vi "Core Read U8 FIFO.vi"(8 "error in (no error)":errorcluster, 9 "Timeout (ms)":i32, 11 "CIFFIFO in":refnum<class "CIF_Iceoryx_PCAP_Universal.lvclass">) -> (0 "error out":errorcluster, 1 "timed out?":bool, 3 "CIFFIFO out":refnum<class "CIF_Iceoryx_PCAP_Universal.lvclass">)   [LabVIEW 2021, in "CIF_Iceoryx_PCAP_Universal.lvclass"]
uses:
  CIF_Iceoryx_PCAP_Universal.lvclass
  D:/dev/Packages/CIF_Channels_Core/src/CIFChannels/CIFChannels.lvclass
  ChannelCommon/typedef/Channel State.ctl
  ChannelCommon/typedef/Direction.ctl
  CIFChannels/CIFChannels.lvclass/CIFChannels.ctl
  CIF_Iceoryx_PCAP_Universal.lvclass/CIF_Iceoryx_PCAP_Universal.ctl
  <vilib>/CIF Foundation/CIF Utilities/Statistics/I64/Stats_I64_CIF_U.lvclass/Stats_I64_CIF_U.ctl
  CIFChannels/Accessors/Write FIFO Header.vi
  CIFChannels/Accessors/Read FIFO Header.vi
  e703c505-0034-46a9-8989-21c0de27793f.vi
  768488f4-e6df-4560-a449-a64b33b49031.vi
  CIFChannels/Accessors/Read Channel State.vi
  CIFChannels/Accessors/Read Direction.vi
  <vilib>/CIF Foundation/CIF Iceoryx/SubVIs/Get Path.vi
  <vilib>/CIF Foundation/CIF Iceoryx/SubVIs/Convert Error.vi
  <vilib>/CIF Foundation/CIF Iceoryx/Refnum/CIF Subscriber from Refnum.vi
  <vilib>/CIF Foundation/CIF Utilities/Statistics/I64/X1 minus X0.vi
  <vilib>/CIF Foundation/CIF Utilities/Time/System Time/Get System Time.vi
  <vilib>/CIF Foundation/CIF Utilities/Statistics/I64/X1 minus X0.vi/dfabcf33-0dbc-4041-80a5-3dc0c86d2989.vi
  <vilib>/CIF Foundation/CIF Utilities/Statistics/I64/X1 minus X0.vi/dfabcf33-0dbc-4041-80a5-3dc0c86d2989.vi/9eb60a9a-770f-4d2d-8b3f-8465c267ecc9.vi
  <vilib>/CIF Foundation/CIF Iceoryx/SubVIs/Convert Error Core.vi
  ChannelCommon/ChannelCommon.lvlib
  CIFChannels/CIFChannels.lvclass
  <vilib>/CIF Foundation/CIF Iceoryx/Iceoryx.lvlib
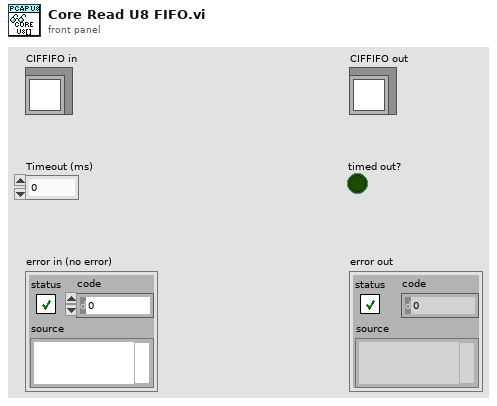
[diagram p1: front panel]
types:
  T1 = typedef "ChannelCommon.lvlib/Channel State.ctl" = enum8{"Creating", "Disconnected", "Connecting", "Connected", "Destroyed"}
  T2 = typedef "ChannelCommon.lvlib/Direction.ctl" = enum8{"Publisher", "Subscriber"}
  T3 = typedef "Iceoryx.lvlib/CIF Subscriber Refnum.ctl" = cluster{"refnum":u64, "CIF Sub":enum8{"cifsub"}}
  T4 = typedef "Iceoryx.lvlib/CIF Channel Header.ctl" = cluster{"Length":u64, "T0":i64, "T_Out":i64, "T_Tx":i64, "Ctr":u64, "ClockID":u8}
  T5 = typedef "ChannelCommon.lvlib/FIFO Header.ctl" = cluster{"Length":u64, "T0":i64, "T_Out":i64, "T_Tx":i64, "Ctr":u64, "ClockID":u8}
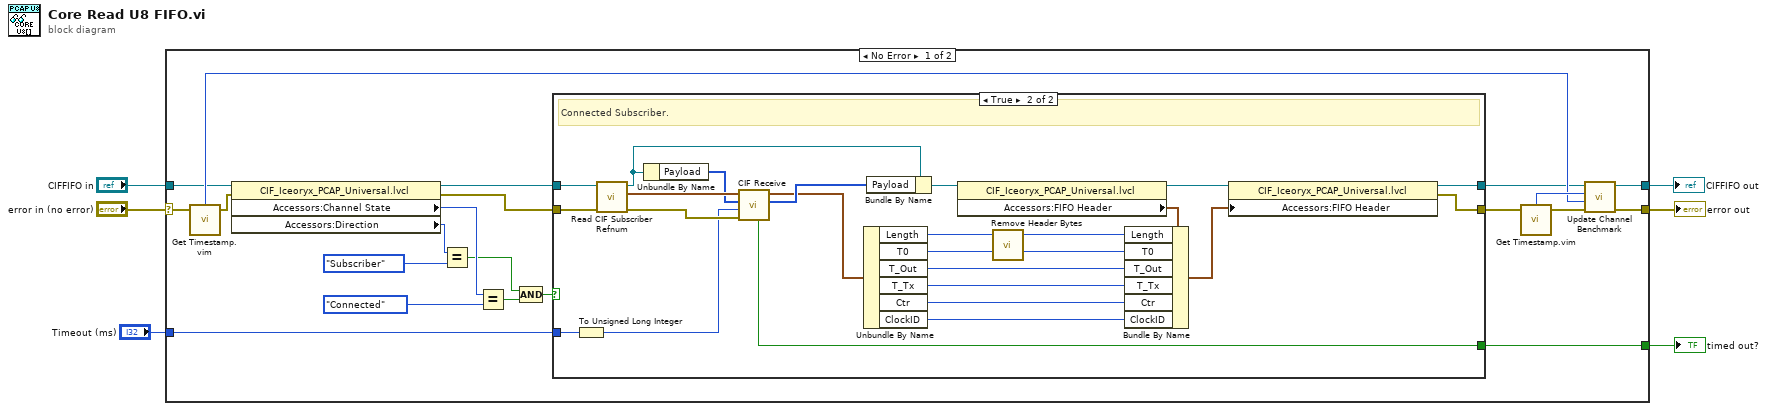
[diagram p0: block diagram]
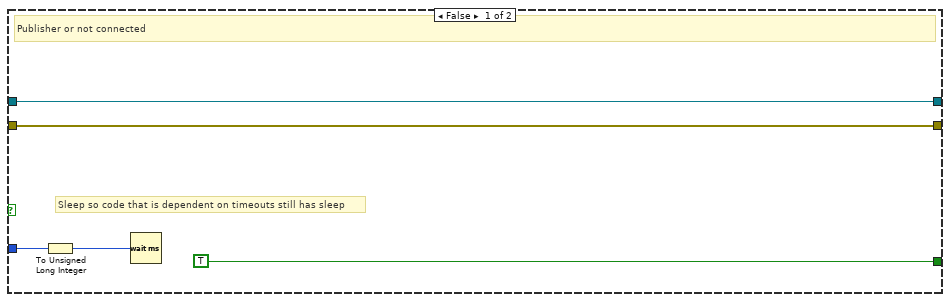
[diagram p2: hidden frame]
diagram:
  n1 = case shown="No Error" "error in (no error)" {
    selector: "error in (no error)" -> [w9 w58]
    tunnel: [w15 w58] -> w1
    tunnel: [w16 w57] -> w2
    tunnel: "CIFFIFO in" -> [w8 w57]
    tunnel: [w27 _] -> w3
    tunnel: "Timeout (ms)" -> [w17 _]
    frame No Error {
      n2 = call "Get Timestamp.vim"("Anything in"=w9) -> ("Time (ns)"=w13:i64, "Anything out"=w7:errorcluster)  [unwired: 2 in]
      n3 = property class="CIF_Iceoryx_PCAP_Universal.lvcl"(reference=w8, error in=w7) -> (reference out=w26:refnum<class "CIF_Iceoryx_PCAP_Universal.lvclass">, error out=w25:errorcluster, "Accessors:Channel State"=w22:T1, "Accessors:Direction"=w24:T2)
      n4 = Equal?(x=w24, y=Direction."Subscriber") -> (x = y?=w18:bool)
      n5 = Equal?(x=w22, y=Channel_State."Connected") -> (x = y?=w20:bool)
      n6 = Compound Arithmetic op=AND(w18, w20) -> (w19:bool)
      n7 = case shown="True" w19 {
        tunnel: [TRUE ("timeout out") w49] -> w27
        tunnel: w25 -> [w31 w56]
        tunnel: w26 -> [w32 w53]
        tunnel: [w32 w36] -> w11
        tunnel: [w31 w35] -> w10
        tunnel: w17 -> [w29 w51]
        frame False {
          # "Sleep so code that is dependent on timeouts still has sleep"
          # "Publisher or not connected"
          n8 = To Unsigned Long Integer(number=w29) -> (unsigned 32bit integer=w28:u32)
          n9 = Wait (ms)(milliseconds to wait=w28) -> ()  [unwired: 1 out]
        }
        frame True {
          # "Connected Subscriber."
          n10 = To Unsigned Long Integer(number=w51) -> (unsigned 32bit integer=w50:u32)
          n11 = call "Read CIF Subscriber Refnum.vi"("error in (no error)"=w56, "CIF_Iceoryx_PCAP_Universal in"=w53) -> ("error out"=w54:errorcluster, "CIF Subscriber Refnum"=w55:T3, "CIF_Iceoryx_PCAP_Universal out"=w48:refnum<class "CIF_Iceoryx_PCAP_Universal.lvclass">)  [unwired: 7 in]
          n12 = Unbundle By Name(w48) -> ("Payload"=w52:u8[])
          n13 = call <vilib>:"CIF Receive.vi"("error in (no error)"=w54, "Timoeut ms"=w50, "Data In"=w52, "Subscriber Reference"=w55) -> ("Data Out"=w47:u8[], "CIF Channel Header"=w44:T4, "Timeout"=w49:bool)  [unwired: 2 in, 3 out]
          n14 = Unbundle By Name(w44) -> ("Length"=w34:u64, "T0"=w43:i64, "T_Out"=w42:i64, "T_Tx"=w41:i64, "Ctr"=w40:u64, "ClockID"=w39:u8)
          n15 = Bundle By Name(cluster=w48, "Payload"=w47) -> (w46:refnum<class "CIF_Iceoryx_PCAP_Universal.lvclass">)
          n16 = property class="CIF_Iceoryx_PCAP_Universal.lvcl"(reference=w46) -> (reference out=w37:refnum<class "CIF_Iceoryx_PCAP_Universal.lvclass">, "Accessors:FIFO Header"=w45:T5)  [unwired: 1 in, 1 out]
          n17 = call "Remove Header Bytes.vi"("Bytes/Msg with header"=w34) -> ("Bytes/Msg without header"=w33:u64)  [unwired: 3 in]
          n18 = Bundle By Name(cluster=w45, "Length"=w33, "T0"=w43, "T_Out"=w42, "T_Tx"=w41, "Ctr"=w40, "ClockID"=w39) -> (w38:T5)
          n19 = property class="CIF_Iceoryx_PCAP_Universal.lvcl"(reference=w37, "Accessors:FIFO Header"=w38) -> (reference out=w36:refnum<class "CIF_Iceoryx_PCAP_Universal.lvclass">, error out=w35:errorcluster)  [unwired: 1 in]
        }
      }
      n20 = call "Get Timestamp.vim"("Anything in"=w10) -> ("Time (ns)"=w14:i64, "Anything out"=w12:errorcluster)  [unwired: 2 in]
      n21 = call "Update Channel Benchmark.vi"("error in (no error)"=w12, "X0"=w13, "X1"=w14, "CIFChannels in"=w11) -> ("error out"=w15:errorcluster, "CIFChannels out"=w16:refnum<class "CIF_Iceoryx_PCAP_Universal.lvclass">)  [unwired: 6 in]
    }
    frame Error {
    }
  }
  "error out" <- w1
  "timed out?" <- w3
  "CIFFIFO out" <- w2
